vi "PicoScope2000RunBlock.vi"(5 "Buffer and Transfer Settings":T1 {"Down-Sample Mode" items=["RAW none", "None", "Aggregate", "Decimate", "Average"]; "Down Sample Ratio" step=1; "Samples" format="%_6p"}, 7 "Acquisition Settings":T2 {"postTriggerSamples" format="%_6p"; "preTriggerSamples" format="%_6p"}, 8 "error in (no error)":errorcluster, 11 "handle in":i16) -> (0 "error out":errorcluster, 3 "handle out":i16, 4 "timeIndisposedMs":dbl, 6 "Total Requested Samples":u64)   [LabVIEW 2009]
doc: "Calls ps5000aRunBlock"
uses:
  ps2000.dll
  shared/Acquisition Settings.ctl
  shared/Buffer and Transfer Settings.ctl
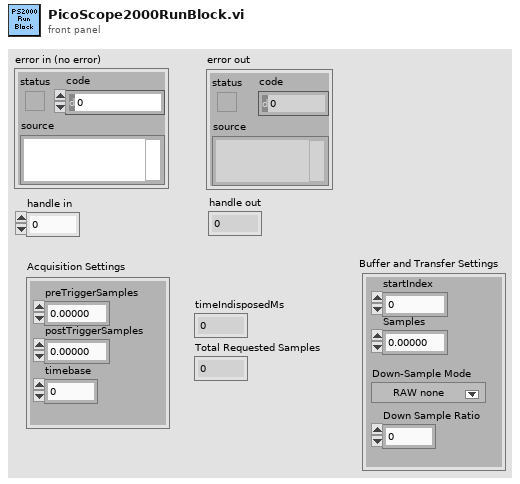
[diagram p1: front panel]
types:
  T1 = typedef "Buffer and Transfer Settings.ctl" = cluster{"startIndex":u64, "Samples":u64, "Down Sample Ratio":u64, "Down-Sample Mode":u32}
  T2 = typedef "Acquisition Settings.ctl" = cluster{"preTriggerSamples":u64, "postTriggerSamples":u64, "timebase":u32}
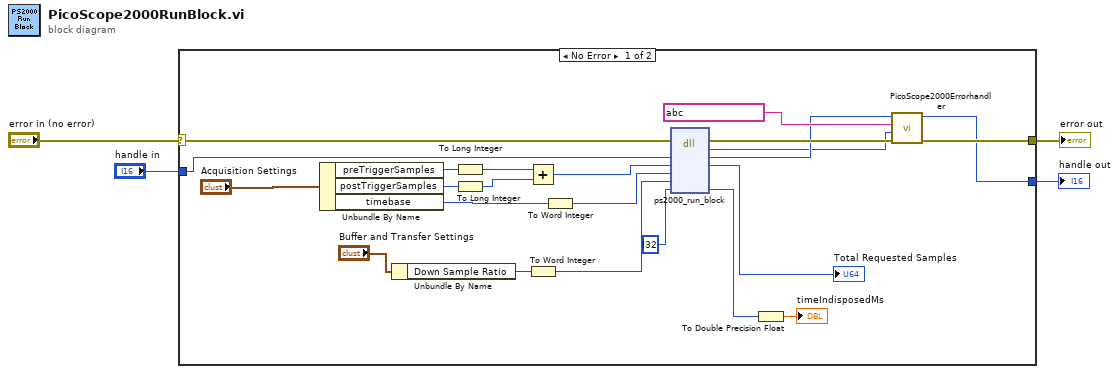
[diagram p0: block diagram]
diagram:
  n1 = case shown="No Error" "error in (no error)" {
    selector: "error in (no error)" -> [w26 w29]
    tunnel: [w10 w29] -> w2
    tunnel: "handle in" -> [w25 w28]
    tunnel: [w6 w28] -> w3
    frame #0 {
      n2 = Unbundle By Name("Acquisition Settings") -> ("preTriggerSamples"=w24:u64, "postTriggerSamples"=w22:u64, "timebase"=w23:u32)
      n3 = Unbundle By Name("Buffer and Transfer Settings") -> ("Down Sample Ratio"=w12:u64)
      n4 = To Long Integer(number=w24) -> (32bit integer=w20:i32)
      n5 = To Long Integer(number=w22) -> (32bit integer=w21:i32)
      n6 = Add(x=w20, y=w21) -> (x+y=w19:i32)
      n7 = To Word Integer(number=w12) -> (16bit integer=w11:i16)
      n8 = To Word Integer(number=w23) -> (16bit integer=w18:i16)
      n9 = dll-call lib="PS2000.dll" fn="ps2000_run_block"(error in=w26, "handle"=w25, "no_of_samples"=w19, "timebase"=w18, "oversample"=w11, "time_indisposed_ms"=i32 ?) -> (error out=w9:errorcluster, "return type"=w5:i16, "handle"=w7:i16, "no_of_samples"=→"Total Requested Samples":i32, "time_indisposed_ms"=w14:i32)  [unwired: 4 in, 1 out]
      n10 = To Double Precision Float(number=w14) -> (double precision float=→"timeIndisposedMs":dbl)
      n11 = call "PicoScope2000Errorhandler.vi"("Handle in"=w7, "API function"=string ? ("source"), "Return"=w5, "error in (no error)"=w9) -> ("Handle out"=w6:i16, "error out"=w10:errorcluster)  [unwired: 5 in]
    }
    frame #1 {
    }
  }
  "error out" <- w2
  "handle out" <- w3
